vi "Read.vi"(8 "error in (no error)":errorcluster, 11 "AnalogInput in":refnum<class "AnalogInput.lvclass">) -> (0 "error out":errorcluster, 2 "Data Out":dbl, 3 "AnalogInput out":refnum<class "AnalogInput.lvclass">)   [LabVIEW 2021, in "AnalogInput.lvclass"]
uses:
  AnalogInput.lvclass
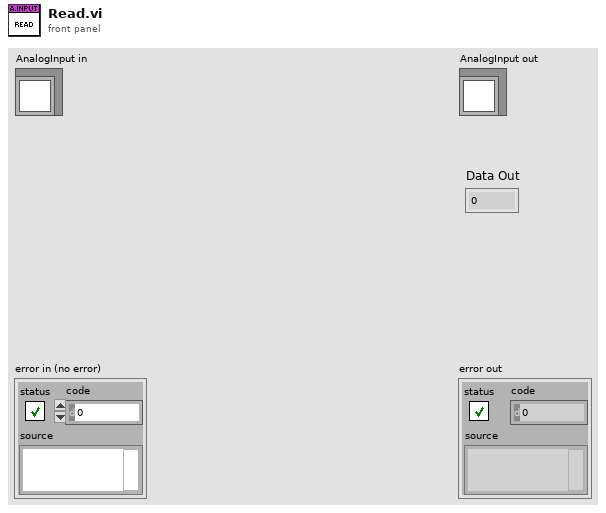
[diagram p1: front panel]
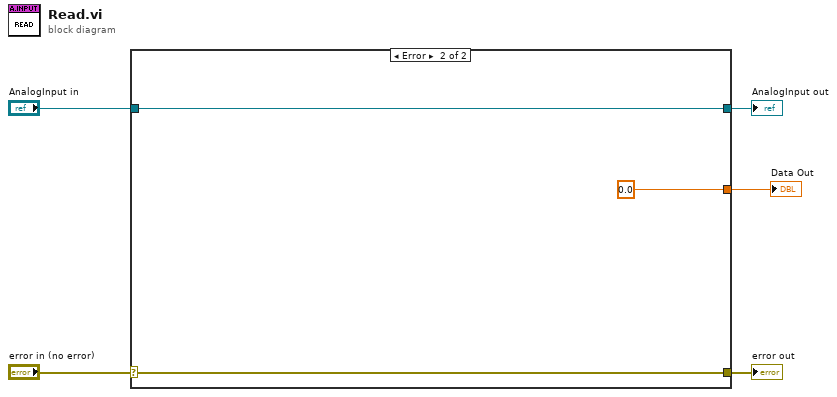
[diagram p0: block diagram]
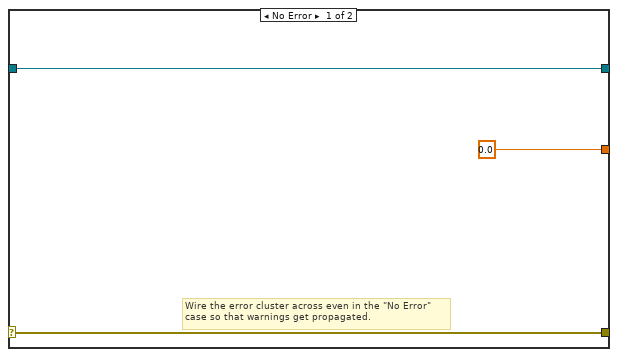
[diagram p2: hidden frame]
diagram:
  n1 = case shown="Error" "error in (no error)" {
    selector: "error in (no error)" -> [w7 w11]
    tunnel: [w7 w11] -> w4
    tunnel: [w8 w10] -> w2
    tunnel: "AnalogInput in" -> [w8 w10]
    tunnel: [0.0 ("Data Out") 0.0 ("Data Out")] -> w1
    frame No Error {
      # "Wire the error cluster across even in the \"No Error\"\ncase so that warnings get propagated."
    }
    frame Error {
    }
  }
  "error out" <- w4
  "AnalogInput out" <- w2
  "Data Out" <- w1
